vi "Create Job.vi"(6 "JobReport type":refnum<class "JobReport.lvclass">, 7 "Job Name":string, 8 "error in (no error)":errorcluster, 11 "Job in":refnum<class "Job.lvclass">) -> (0 "error out":errorcluster, 3 "Job":refnum<class "Job.lvclass">)   [LabVIEW 2013, in "openCronJob.lvlib" / "Job.lvclass"]
uses:
  Job.lvclass
  JobReport/JobReport.lvclass
  Job.lvclass/Job.ctl
  Job Started -- cluster.ctl
  Job Update -- cluster.ctl
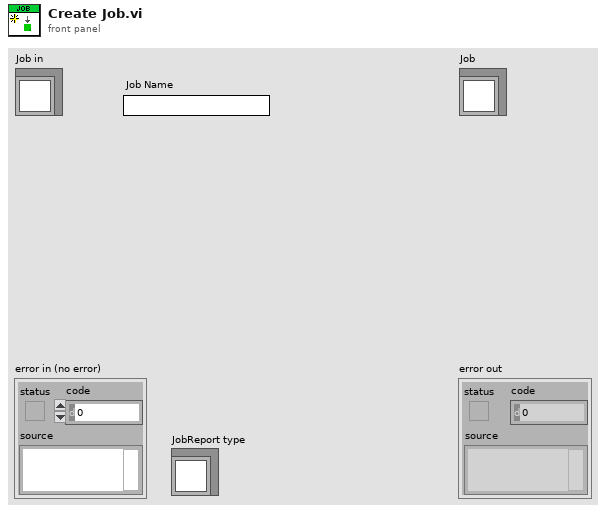
[diagram p1: front panel]
types:
  T1 = typedef "openCronJob.lvlib/Job.lvclass/Job Update -- cluster.ctl" = cluster{"Name":string, "GUID":string, "Time Stamp":timestamp, "Status Message":string, "% Complete":dbl}
  T2 = typedef "openCronJob.lvlib/Job.lvclass/Job Started -- cluster.ctl" = cluster{"Name":string, "GUID":string, "Time Stamp":timestamp}
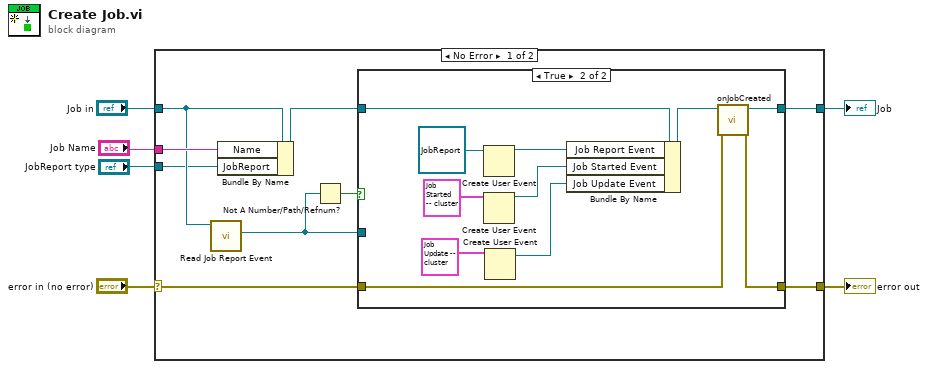
[diagram p0: block diagram]
diagram:
  n1 = case shown="No Error" "error in (no error)" {
    selector: "error in (no error)" -> [w11 w30]
    tunnel: [w10 w30] -> w5
    tunnel: [w15 w29] -> w3
    tunnel: "Job in" -> [w9 w29]
    tunnel: "Job Name" -> [w13 _]
    tunnel: "JobReport type" -> [w7 _]
    frame No Error {
      n2 = call "Read Job Report Event.vi"("Job in"=w9) -> ("Job Report Event"=w8:refnum<user-event>)  [unwired: 7 in, 3 out]
      n3 = Bundle By Name(cluster=w9, "Name"=w13, "JobReport"=w7) -> (w12:refnum<class "Job.lvclass">)
      n4 = Not A Number/Path/Refnum?(number/path/refnum=w8) -> (NaN/Path/Refnum?=w14:bool)
      n5 = case shown="True" w14 {
        tunnel: [w17 w26] -> w15
        tunnel: w12 -> [w17 w22]
        tunnel: w8 -> [_ _]
        tunnel: w11 -> [w16 w25]
        tunnel: [w16 w24] -> w10
        frame False {
          # "Job Report Event already exists"
        }
        frame True {
          n6 = Create User Event(user event datatype=refnum<class "JobReport.lvclass"> refnum ("openCronJob.lvlib:JobReport.lvclass")) -> (user event=w28:refnum<user-event>)  [unwired: 1 in, 1 out]
          n7 = Create User Event(user event datatype=T2 {"Name"="", "GUID"="", "Time Stamp"=timestamp(0 s since 1904-01-01)} ("Job Started")) -> (user event=w20:refnum<user-event>)  [unwired: 1 in, 1 out]
          n8 = Create User Event(user event datatype=T1 {"Name"="", "GUID"="", "Time Stamp"=timestamp(0 s since 1904-01-01), "Status Message"="", "% Complete"=nan} ("Job Update")) -> (user event=w18:refnum<user-event>)  [unwired: 1 in, 1 out]
          n9 = Bundle By Name(cluster=w22, "Job Report Event"=w28, "Job Started Event"=w20, "Job Update Event"=w18) -> (w27:refnum<class "Job.lvclass">)
          n10 = call-dynamic "onJobCreated.vi"("error in (no error)"=w25, "Job in"=w27) -> ("error out"=w24:errorcluster, "Job out"=w26:refnum<class "Job.lvclass">)  [unwired: 8 in]
        }
      }
    }
    frame Error {
    }
  }
  "error out" <- w5
  "Job" <- w3
